vi "Create Basic Response.vi"   [LabVIEW 2020]
uses:
  lv-http-util/HTTP Utils/Response/Response.lvclass
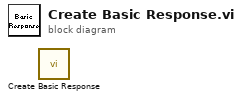
[diagram p0: block diagram]
diagram:
  n1 = call "Create Basic Response.vi"() -> ()  [unwired: 10 in, 2 out]
